vi "Get Tasks for Project.vi"(7 "Project Store in":refnum<class "Project Store.lvclass">, 8 "error in (no error)":errorcluster, 10 "include inactive?":bool, 11 "Project ID":string) -> (0 "error out":errorcluster, 3 "Tasks":T1, 5 "Project Store out":refnum<class "Project Store.lvclass">)   [LabVIEW 2024, in "Project Store.lvclass"]
doc: "Returns the tasks that belong to the given project, sorted by Sort Order. Inactive tasks are left out unless include inactive? is TRUE.\n\nGenerated by: Claude"
uses:
  Project Store.lvclass
  Project Store.lvclass/Project Store.ctl
  Rows/Task.ctl
  Rows/Task List.ctl
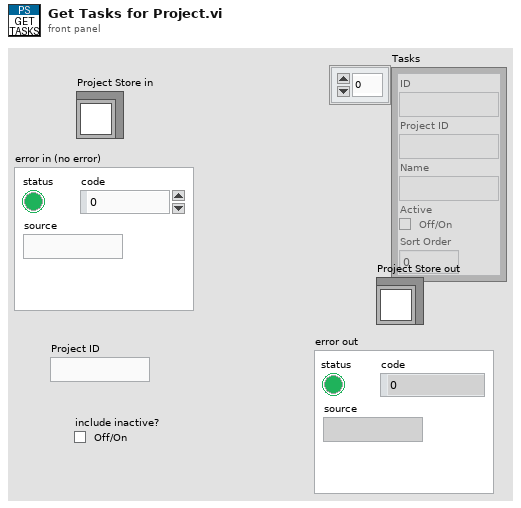
[diagram p1: front panel]
types:
  T1 = typedef "Task List.ctl" = T2[]
  T2 = typedef "Task.ctl" = cluster{"ID":string, "Project ID":string, "Name":string, "Active":bool, "Sort Order":i32}
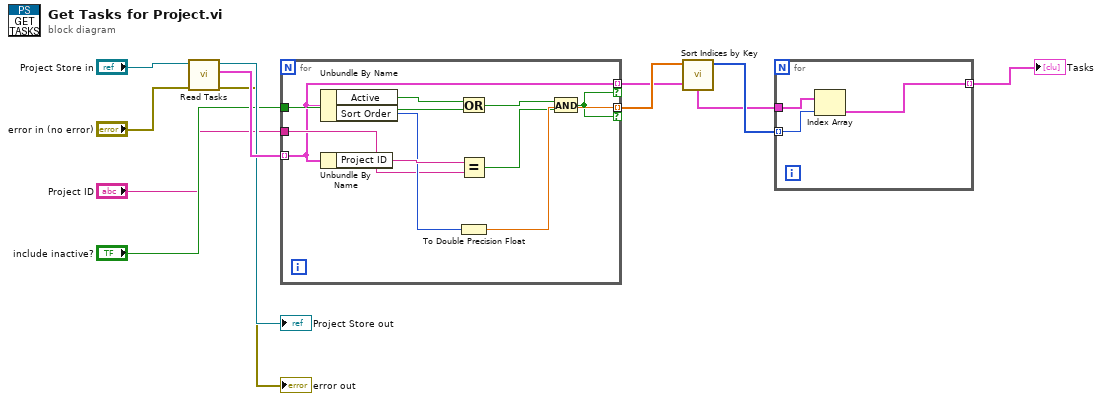
[diagram p0: block diagram]
diagram:
  n1 = call-dynamic "Read Tasks.vi"("error in (no error)"="error in (no error)", "Project Store in"="Project Store in") -> ("error out"=→"error out":errorcluster, "Task List"=w7:T1, "Project Store out"=→"Project Store out":refnum<class "Project Store.lvclass">)  [unwired: 7 in]
  n2 = for {
    tunnel: "include inactive?" -> [w13]
    tunnel: "Project ID" -> [w14]
    tunnel: w7 -> [w12] mode=indexing
    tunnel: [w12] -> w8 mode=indexing if=w20
    tunnel: [w21] -> w9 mode=indexing if=w20
    n3 = Unbundle By Name(w12) -> ("Active"=w15:bool, "Sort Order"=w16:i32)
    n4 = Unbundle By Name(w12) -> ("Project ID"=w18:string)
    n5 = Or(x=w15, y=w13) -> (x .or. y?=w17:bool)
    n6 = Equal?(x=w18, y=w14) -> (x = y?=w19:bool)
    n7 = To Double Precision Float(number=w16) -> (double precision float=w21:dbl)
    n8 = And(x=w17, y=w19) -> (x .and. y?=w20:bool)
  }
  n9 = call "Sort Indices by Key.vi"("Keys"=w9) -> ("Sorted Indices"=w10:i32[])  [unwired: 9 in, 1 out]
  n10 = for {
    tunnel: w8 -> [w23]
    tunnel: w10 -> [w22] mode=indexing
    tunnel: [w24] -> w11 mode=indexing
    n11 = Index Array(array=w23, index=w22) -> (element=w24:T2)
  }
  "Tasks" <- w11
